vi "Build RT Data Cluster.vi"(0 "Device Reference in":T1 format="%.0x", 2 "RT Data in":T2={"Device ref"=0, "Scan Period (uSec)"=10000, "Device Channels"={"Status"={"BD Refs"=[], "Length"=0, "FIFO Index"=0, "Data"=[]}, "Command"={"BD Refs"=[], "Data"=[], "Length"=0, "FIFO Index"=0}}, "Local Chassis"=[], "EtherCAT Masters"=[], "Async"={"Status"=refnum, "Command"=refnum, "Input FIFO"=refnum, "Input FIFO buffer"=[], "Output FIFO"=refnum, "Output FIFO buffer"=[], "Async VI Ref"=refnum}, "ECAT Reconfig"={"Reconfig Module Found"=FALSE, "VI Ref"=refnum, "Status"=refnum}, "Device Error"={"status"=FALSE, "code"=0, "source"=""}, "DeviceName"="", "PCLSync?"=FALSE} {"Device Channels"."Status"."BD Refs"."Data Reference" format="%.0x"; "Device Channels"."Command"."BD Refs"."Data Reference" format="%.0x"; "Local Chassis"."FPGA"."VS ref" format="%.0x"; "Local Chassis"."RSI Modules"."VS ref" format="%.0x"; "Local Chassis"."VS ref" format="%.0x"; "Device ref" format="%.0x"; "EtherCAT Masters"."REM IO ECAT Slaves"."VS ref" format="%.0x"; "EtherCAT Masters"."Generic EtherCAT Slaves"."VS ref" format="%.0x"; "EtherCAT Masters"."VS ref" format="%.0x"; "EtherCAT Masters"."EtherCAT Slaves"."FPGA"."VS ref" format="%.0x"; "EtherCAT Masters"."EtherCAT Slaves"."RSI Modules"."VS ref" format="%.0x"; "EtherCAT Masters"."EtherCAT Slaves"."VS ref" format="%.0x"}, 3 "error in":errorcluster) -> (7 "RT Data out":T2={"Device ref"=0, "Scan Period (uSec)"=10000, "Device Channels"={"Status"={"BD Refs"=[], "Length"=0, "FIFO Index"=0, "Data"=[]}, "Command"={"BD Refs"=[], "Data"=[], "Length"=0, "FIFO Index"=0}}, "Local Chassis"=[], "EtherCAT Masters"=[], "Async"={"Status"=refnum, "Command"=refnum, "Input FIFO"=refnum, "Input FIFO buffer"=[], "Output FIFO"=refnum, "Output FIFO buffer"=[], "Async VI Ref"=refnum}, "ECAT Reconfig"={"Reconfig Module Found"=FALSE, "VI Ref"=refnum, "Status"=refnum}, "Device Error"={"status"=FALSE, "code"=0, "source"=""}, "DeviceName"="", "PCLSync?"=FALSE} {"Device Channels"."Status"."BD Refs"."Data Reference" format="%.0x"; "Device Channels"."Command"."BD Refs"."Data Reference" format="%.0x"; "Local Chassis"."FPGA"."VS ref" format="%.0x"; "Local Chassis"."RSI Modules"."VS ref" format="%.0x"; "Local Chassis"."VS ref" format="%.0x"; "Device ref" format="%.0x"; "EtherCAT Masters"."REM IO ECAT Slaves"."VS ref" format="%.0x"; "EtherCAT Masters"."Generic EtherCAT Slaves"."VS ref" format="%.0x"; "EtherCAT Masters"."VS ref" format="%.0x"; "EtherCAT Masters"."EtherCAT Slaves"."FPGA"."VS ref" format="%.0x"; "EtherCAT Masters"."EtherCAT Slaves"."RSI Modules"."VS ref" format="%.0x"; "EtherCAT Masters"."EtherCAT Slaves"."VS ref" format="%.0x"})   [LabVIEW 2020, in "SEECD Engine.lvlib"]
uses:
  SEECD Engine.lvlib
  Type Defs/RT Data.ctl
  <vilib>/NI VeriStand/Custom Device API/Custom Device Item Ref.ctl
  Type Defs/Device Channels.ctl
  Type Defs/Output Data.ctl
  <vilib>/NI VeriStand/Custom Device API/Block Data Reference.ctl
  <vilib>/NI VeriStand/Custom Device API/Data Reference.ctl
  Type Defs/Input Data.ctl
  Type Defs/Local Chassis Data.ctl
  Type Defs/RSI Module Data.ctl
  Type Defs/Open Module IOVs.ctl
  Includes/Modules.lvlibp/RSI Module/RSI Module.lvclass
  Includes/Modules.lvlibp/RSI Module/Module Models.ctl
  Includes/Modules.lvlibp/RSI Module/Channel Type.ctl
  Type Defs/Module Config Data.ctl
  Type Defs/Mixed IO.ctl
  Type Defs/FPGA Data.ctl
  Type Defs/UDV Data.ctl
  Shared/Type Defs/UDV Data Type.ctl
  Shared/Type Defs/FXP Config.ctl
  Type Defs/Mod Size Indexes.ctl
  Type Defs/EtherCAT Master Data.ctl
  Type Defs/EtherCAT Slave Data.ctl
  Type Defs/Generic ECAT Slave RT-Data-Array.ctl
  Type Defs/Generic ECAT Slave Data Cluster.ctl
  Type Defs/Generic ECAT Slave IOV Cluster.ctl
  Type Defs/REM IO ECAT Slave RT-Data-Array.ctl
  Type Defs/REM IO ECAT Slave Data Cluster.ctl
  Type Defs/REM IO ECAT Slave IOV Cluster.ctl
  Type Defs/Async Data.ctl
  Type Defs/Async Status.ctl
  Type Defs/Async State.ctl
  Type Defs/Async Command.ctl
  Type Defs/ECAT Reconfig Data.ctl
  Type Defs/ECAT Reconfig Status.ctl
  Type Defs/ECAT Reconfig State.ctl
  Type Defs/Data Ref FGV Command.ctl
  <vilib>/NIScanEngine/ConfigurableFaults/Fault Desc Control.ctl
  Shared/Globals/Property Strings.vi
  Shared/Globals/RT Globals.vi
  Shared/Globals/String Constants.vi
  <vilib>/NI VeriStand/Custom Device API/Get Item Property (U16).vi
  <vilib>/NI VeriStand/Custom Device API/Get Item Property (U32).vi
  <vilib>/NI VeriStand/Custom Device API/Custom Device API.lvlib
  Shared/SEECD Shared.lvlib
  <vilib>/NI VeriStand/Custom Device Tools/Custom Device Utility Library/Custom Device Utility Library.lvlib
  <vilib>/NIScanEngine/ConfigurableFaults/Config Faults.lvlib
  <vilib>/NI VeriStand/Custom Device API/Get Item Property (Boolean).vi
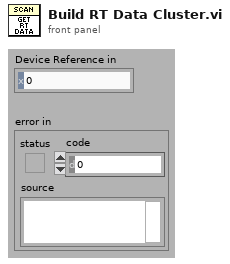
[diagram p1: front panel]
types:
  T1 = typedef "Custom Device API.lvlib/Custom Device Item Ref.ctl" = u64
  T2 = typedef "SEECD Engine.lvlib/RT Data.ctl" = cluster{"Device ref":T1, "Scan Period (uSec)":u32, "Device Channels":T3, "Local Chassis":T8[], "EtherCAT Masters":T20[], "Async":T28, "ECAT Reconfig":T29, "Device Error":errorcluster, "DeviceName":string, "PCLSync?":bool}
  T3 = typedef "SEECD Engine.lvlib/Device Channels.ctl" = cluster{"Status":T4, "Command":T7}
  T4 = typedef "SEECD Engine.lvlib/Output Data.ctl" = cluster{"BD Refs":T5[], "Length":i32, "FIFO Index":i32, "Data":dbl[]}
  T5 = typedef "Custom Device API.lvlib/Block Data Reference.ctl" = cluster{"Data Reference":T6, "Offset":u64, "Length":u64}
  T6 = typedef "Custom Device API.lvlib/Data Reference.ctl" = i32
  T7 = typedef "SEECD Engine.lvlib/Input Data.ctl" = cluster{"BD Refs":T5[], "Data":dbl[], "Length":i32, "FIFO Index":i32}
  T8 = typedef "SEECD Engine.lvlib/Local Chassis Data.ctl" = cluster{"VS ref":T1, "RSI Modules":T9[], "FPGA":T15[], "Input Mod Size Idxs":T19, "Output Modules":i32[], "MixedIO Mod Size Idxs":T19}
  T9 = typedef "SEECD Engine.lvlib/RSI Module Data.ctl" = cluster{"VS ref":T1, "IOV ref":refnum<k21>, "Open Mod refs":T10, "Module DVR":refnum<data-value>, "Slot":u32, "Model":T11, "Channel Type":T12, "EtherCAT?":bool, "CDInput Data":T7, "CDOutput Data":T4, "Module Config Data":T13, "Mixed IO":T14}
  T10 = typedef "SEECD Engine.lvlib/Open Module IOVs.ctl" = cluster{"Analog Read":refnum<k21>, "Digital Read":refnum<k21>, "Analog Write":refnum<k21>, "Digital Write":refnum<k21>}
  T11 = typedef "Modules.lvlibp/RSI Module.lvclass/Module Models.ctl" = enum16{"Empty", "NI 9201", "NI 9203", "NI 9205", "NI 9206", "NI 9207", "NI 9208", "NI 9209", "NI 9210", "NI 9211", "NI 9212", "NI 9213", "NI 9214", "NI 9215", "NI 9216", "NI 9217", "NI 9219", "NI 9220", "NI 9221", "NI 9222", "NI 9223", "NI 9224", "NI 9225", "NI 9226", "NI 9227", "NI 9228", "NI 9229", "NI 9233", "NI 9234", "NI 9235", "NI 9236", "NI 9237", "NI 9239", "NI 9242", "NI 9244", "NI 9253", "NI 9263", "NI 9264", "NI 9265", "NI 9266", "NI 9269", "NI 9344", "NI 9350", "NI 9375", "NI 9401", "NI 9402", "NI 9403", "NI 9411", "NI 9421", "NI 9422", "NI 9423", "NI 9425", "NI 9426", "NI 9435", "NI 9436", "NI 9437", "NI 9472", "NI 9474", "NI 9475", "NI 9476", "NI 9477", "NI 9478", "NI 9481", "NI 9482", "NI 9485"}
  T12 = typedef "Modules.lvlibp/RSI Module.lvclass/Channel Type.ctl" = enum16{"Analog", "Digital"}
  T13 = typedef "SEECD Engine.lvlib/Module Config Data.ctl" = cluster{"Configurable?":bool, "Config Block Data Refs":T5[], "Config Data DVR":refnum<data-value>, "Previous Values":dbl[], "Local Reconfig VI Ref":refnum<vi>}
  T14 = typedef "SEECD Engine.lvlib/Mixed IO.ctl" = cluster{"Input Channel Indices":i32[], "Input Buffer":dbl[]}
  T15 = typedef "SEECD Engine.lvlib/FPGA Data.ctl" = cluster{"VS ref":T1, "IOV ref":refnum<k21>, "FPGA Target":enum16{"Local", "EtherCAT"}, "Product Code":u32, "Bitfile Signature":string, "Bitfile Path (RT)":path, "FPGA Session":u32, "Input Data":T7, "Output Data":T4, "UDVs":cluster{"From FPGA":T16[], "To FPGA":T16[]}}
  T16 = typedef "SEECD Engine.lvlib/UDV Data.ctl" = cluster{"VS ref":T1, "IOV Ref":refnum<k21>, "Name":string, "UDV Data Type":T17, "Supported Type?":bool, "FXP Config":T18, "FXP VI Ref":refnum<vi>}
  T17 = typedef "SEECD Shared.lvlib/UDV Data Type.ctl" = enum16{"Boolean", "Fixed Point", "Int8", "Int16", "Int32", "Int64", "U32 Bit Field", "UInt8", "UInt16", "UInt32", "UInt64", "Other", "DBL", "SGL"}
  T18 = typedef "SEECD Shared.lvlib/FXP Config.ctl" = cluster{"signed":bool, "size":u32, "integersize":i32}
  T19 = typedef "SEECD Engine.lvlib/Mod Size Indexes.ctl" = cluster{"4":i32[], "8":i32[], "16":i32[], "32":i32[], "other":i32[]}
  T20 = typedef "SEECD Engine.lvlib/EtherCAT Master Data.ctl" = cluster{"VS ref":T1, "IOV ref":refnum<k21>, "Master ID":u32, "Cyclic Data Bandwidth":u32, "EtherCAT Slaves":T21[], "Generic EtherCAT Slaves":T22, "REM IO ECAT Slaves":T25}
  T21 = typedef "SEECD Engine.lvlib/EtherCAT Slave Data.ctl" = cluster{"VS ref":T1, "IOV ref":refnum<k21>, "Position Address":u16, "RSI Modules":T9[], "FPGA":T15[], "Input Mod Size Idxs":T19, "Output Modules":i32[], "MixedIO Mod Size Idxs":T19}
  T22 = typedef "SEECD Engine.lvlib/Generic ECAT Slave RT-Data-Array.ctl" = T23[]
  T23 = typedef "SEECD Engine.lvlib/Generic ECAT Slave Data Cluster.ctl" = cluster{"VS ref":T1, "IOV ref":refnum<k21>, "Position Address":u16, "I/O Imput Vars ":T24[], "I/O Output Vars":T24[], "I/O Input Data":T7, "I/O Output Data":T4, "Distributed Clock":bool}
  T24 = typedef "SEECD Engine.lvlib/Generic ECAT Slave IOV Cluster.ctl" = cluster{"VS ref":T1, "IOV Ref":refnum<k21>, "Name":string, "UDV Data Type":T17}
  T25 = typedef "SEECD Engine.lvlib/REM IO ECAT Slave RT-Data-Array.ctl" = T26[]
  T26 = typedef "SEECD Engine.lvlib/REM IO ECAT Slave Data Cluster.ctl" = cluster{"VS ref":T1, "IOV ref":refnum<k21>, "Position Address":u16, "I/O Imput Vars ":T27[], "I/O Output Vars":T27[], "I/O Input Data":T7, "I/O Output Data":T4}
  T27 = typedef "SEECD Engine.lvlib/REM IO ECAT Slave IOV Cluster.ctl" = cluster{"VS ref":T1, "IOV Ref":refnum<k21>, "Name":string, "UDV Data Type":T17, "Scaling Factor":dbl}
  T28 = typedef "SEECD Engine.lvlib/Async Data.ctl" = cluster{"Status":refnum<queue>, "Command":refnum<queue>, "Input FIFO":refnum<k33>, "Input FIFO buffer":dbl[], "Output FIFO":refnum<k33>, "Output FIFO buffer":dbl[], "Async VI Ref":refnum<vi>}
  T29 = typedef "SEECD Engine.lvlib/ECAT Reconfig Data.ctl" = cluster{"Reconfig Module Found":bool, "VI Ref":refnum<vi>, "Status":refnum<queue>}
  T30 = typedef "Config Faults.lvlib/Fault Desc Control.ctl" = cluster{"code":i32, "level or level before threshold":i32, "occurrence threshold":u32, "time window in seconds":u32, "level after threshold":i32}
  T31 = typedef "SEECD Engine.lvlib/Data Ref FGV Command.ctl" = enum16{"Intialize", "Get", "Update"}
  T32 = typedef "Fault.ctl" = cluster{"code":i32, "level":i32, "first reported time":timestamp, "number reported":u32}
  T33 = typedef "Custom Device API.lvlib/Custom Device Channel.ctl" = cluster{"Type":T34, "Units":string, "Default Value":dbl, "Faultable":bool, "Scalable":bool}
  T34 = typedef "Custom Device API.lvlib/Custom Device Channel Type.ctl" = enum16{"Input", "Output"}
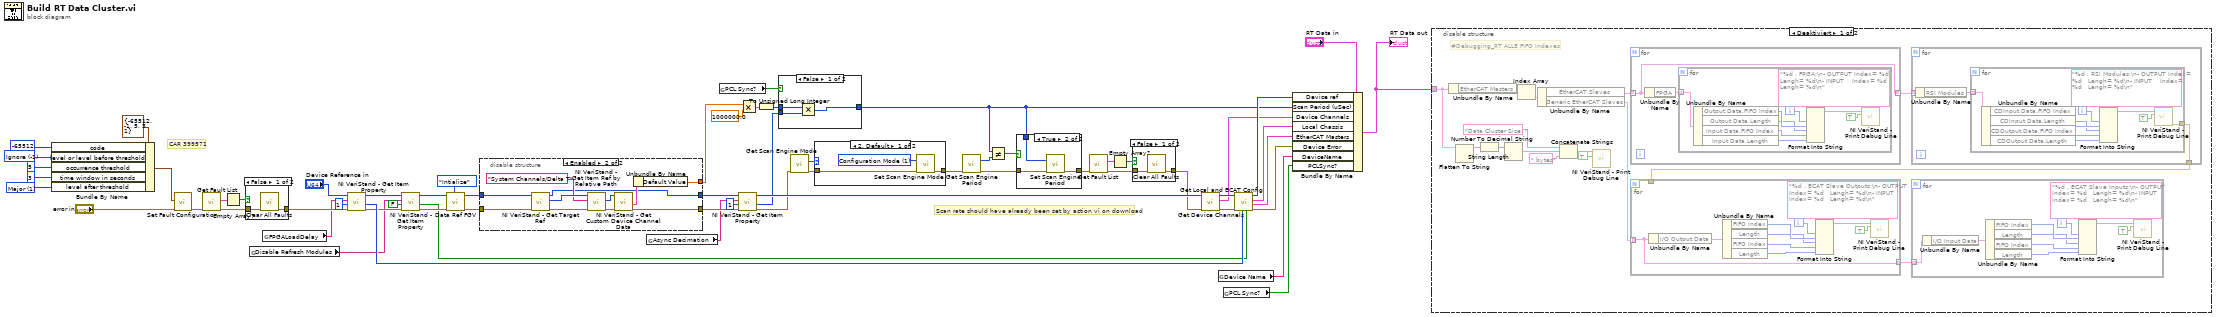
[diagram p0: block diagram]
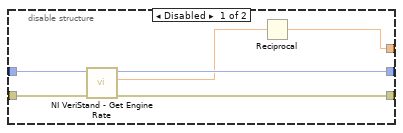
[diagram p7: hidden frame]
diagram:
  w19 = -1 items=["Ignore"=-1, "Minor"=0, "Major"=1] ("level or level before threshold")
  w22 = 1 items=["Ignore"=-1, "Minor"=0, "Major"=1] ("level after threshold")
  # "CAR 399571"
  # "Scan rate should have already been set by action vi on download"
  n1 = Bundle By Name(cluster=T30 {"code"=-65512, "level or level before threshold"=-1, "occurrence threshold"=5, "time window in seconds"=3, "level after threshold"=1} ("fault configuration"), "code"=-65512, "level or level before threshold"=w19, "occurrence threshold"=u32 5, "time window in seconds"=u32 3, "level after threshold"=w22) -> (w23:T30)
  n2 = call <vilib>:"Set Fault Configuration.vi"("error in (no error)"="error in", "fault configuration"=w23) -> ("error out"=w17:errorcluster)  [unwired: 7 in]
  n3 = call <vilib>:"Get Fault List.vi"("error in (no error)"=w17) -> ("error out"=w28:errorcluster, "fault list"=w26:T32[])  [unwired: 9 in]
  n4 = Empty Array?(array=w26) -> (empty?=w27:bool)
  n5 = case shown="False" w27 {
    tunnel: w28 -> [w64 w65]
    tunnel: [w63 w65] -> w25
    frame False {
      n6 = call <vilib>:"Clear All Faults.vi"("error in (no error)"=w64) -> ("error out"=w63:errorcluster)  [unwired: 10 in]
    }
    frame True {
    }
  }
  n7 = global read "Property Strings.vi" "Disable Refresh Modules"() -> (w3:string)
  n8 = global read "Property Strings.vi" "FPGALoadDelay"() -> (w12:string)
  n9 = call-poly <vilib>:"NI VeriStand - Get Item Property.vi"("error in (no error)"=w25, "Default Value"=u16 1, "Property Name"=w12, "Item Ref in"="Device Reference in") -> ("error out"=w7:errorcluster, "Value"=w9:u16, "Item Ref out"=w5:T1)  [unwired: 4 in, 1 out]
  n10 = call-poly <vilib>:"NI VeriStand - Get Item Property.vi"("error in (no error)"=w7, "Default Value"=FALSE, "Property Name"=w3, "Item Ref in"=w5) -> ("error out"=w6:errorcluster, "Value"=w1:bool, "Item Ref out"=w4:T1)  [unwired: 4 in, 1 out]
  n11 = call "Data Ref FGV.vi"("Command"=Data_Ref_FGV_Command."Intialize", "error in (no error)"=w6, "Device Ref in"=w4) -> ("error out"=w62:errorcluster, "Device Ref out"=w61:T1)  [unwired: 5 in, 2 out]
  n12 = disable-structure shown="Enabled" {
    disable-tunnel: [w66 w73] -> w56
    disable-tunnel: [w71 w72] -> w50
    disable-tunnel: [w70 w74] -> w51
    disable-tunnel: w62 -> [w69 w81]
    disable-tunnel: w61 -> [w68 w82]
    frame Disabled {
      n13 = call <vilib>:"NI VeriStand - Get Engine Rate.vi"("error in (no error)"=w69, "Item Ref in"=w68) -> ("error out"=w71:errorcluster, "Rate (Hz)"=w67:dbl, "Item Ref out"=w70:T1)  [unwired: 7 in]
      n14 = Reciprocal(x=w67) -> (1/x=w66:dbl)
    }
    frame Enabled {
      n15 = call <vilib>:"NI VeriStand - Get Target Ref.vi"("error in"=w81, "Item Ref in"=w82) -> ("error out"=w79:errorcluster, "Target Ref"=w80:T1, "Item Ref out"=w74:T1)  [unwired: 6 in, 1 out]
      n16 = call <vilib>:"NI VeriStand - Get Item Ref by Relative Path.vi"("error in"=w79, "Relative Item Path"="System Channels/Delta T", "Section Ref in"=w80) -> ("error out"=w76:errorcluster, "Item Ref"=w77:T1)  [unwired: 5 in, 2 out]
      n17 = call <vilib>:"NI VeriStand - Get Custom Device Channel Data.vi"("error in (no error)"=w76, "Channel Ref in"=w77) -> ("error out"=w72:errorcluster, "Channel"=w75:T33)  [unwired: 4 in, 4 out]
      n18 = Unbundle By Name(w75) -> ("Default Value"=w73:dbl)
    }
  }
  n19 = global read "Property Strings.vi" "Async Decimation"() -> (w48:string)
  n20 = global read "RT Globals.vi" "PCL Sync?"() -> (w45:bool)
  n21 = call-poly <vilib>:"NI VeriStand - Get Item Property.vi"("error in (no error)"=w50, "Default Value"=u32 1, "Property Name"=w48, "Item Ref in"=w51) -> ("error out"=w36:errorcluster, "Value"=w46:u32, "Item Ref out"=w49:T1)  [unwired: 4 in, 1 out]
  n22 = Multiply(x=w56, y=1000000.0) -> (x*y=w30:dbl)
  n23 = To Unsigned Long Integer(number=w30) -> (unsigned 32bit integer=w29:u32)
  n24 = case shown="False" w45 {
    tunnel: w29 -> [w85 w86]
    tunnel: w46 -> [w84 _]
    tunnel: [w83 w86] -> w31
    frame False {
      n25 = Multiply(x=w85, y=w84) -> (x*y=w83:u32)
    }
    frame True {
    }
  }
  n26 = call <vilib>:"Get Scan Engine Mode.vi"("error in (no error)"=w36) -> ("error out"=w38:errorcluster, "mode"=w37:i32)  [unwired: 9 in]
  n27 = case shown="2, Default" w37 {
    tunnel: w38 -> [w88 w90]
    tunnel: [w87 w90] -> w35
    frame 2, Default {
      w89 = 1 items=["Configuration Mode"=1, "Active Mode"=2] ("mode (Active Mode)")
      n28 = call <vilib>:"Set Scan Engine Mode.vi"("mode (Active Mode)"=w89, "error in (no error)"=w88) -> ("error out"=w87:errorcluster)  [unwired: 13 in]
    }
    frame 1 {
    }
  }
  n29 = call <vilib>:"Get Scan Engine Period.vi"("error in (no error)"=w35) -> ("scan period (uSec)"=w34:u32, "error out"=w32:errorcluster)  [unwired: 13 in]
  n30 = Not Equal?(x=w31, y=w34) -> (x != y?=w33:bool)
  n31 = case shown="True" w33 {
    tunnel: [w91 w94] -> w40
    tunnel: w32 -> [w91 w93]
    tunnel: w31 -> [_ w92]
    frame False {
    }
    frame True {
      n32 = call <vilib>:"Set Scan Engine Period.vi"("scan period (uSec)"=w92, "error in (no error)"=w93) -> ("error out"=w94:errorcluster)  [unwired: 13 in]
    }
  }
  n33 = call <vilib>:"Get Fault List.vi"("error in (no error)"=w40) -> ("error out"=w43:errorcluster, "fault list"=w41:T32[])  [unwired: 9 in]
  n34 = Empty Array?(array=w41) -> (empty?=w42:bool)
  n35 = case shown="False" w42 {
    tunnel: w43 -> [w96 w97]
    tunnel: [w95 w97] -> w39
    frame False {
      n36 = call <vilib>:"Clear All Faults.vi"("error in (no error)"=w96) -> ("error out"=w95:errorcluster)  [unwired: 10 in]
    }
    frame True {
    }
  }
  n37 = call "Get Device Channels.vi"("error in"=w39, "Device Reference in"=w49) -> ("error out"=w54:errorcluster, "Device Channels"=w52:T3, "Device Reference out"=w53:T1)  [unwired: 7 in]
  n38 = global read "String Constants.vi" "Device Name"() -> (w15:string)
  n39 = global read "RT Globals.vi" "PCL Sync?"() -> (w14:bool)
  n40 = call "Get Local and ECAT Config.vi"("Disable Refresh Modules"=w1, "fpga wait (s)"=w9, "error in (no error)"=w54, "Device Reference in"=w53) -> ("error out"=w10:errorcluster, "ECAT Masters"=w44:T20[], "Local Chassis"=w60:T8[], "Device Reference out"=w58:T1)  [unwired: 4 in]
  n41 = Bundle By Name(cluster="RT Data in", "Device ref"=w58, "Scan Period (uSec)"=w31, "Device Channels"=w52, "Local Chassis"=w60, "EtherCAT Masters"=w44, "Device Error"=w10, "DeviceName"=w15, "PCLSync?"=w14) -> (w8:T2)
  "RT Data out" <- w8
  n42 = disable-structure shown="Deaktiviert" {
    disable-tunnel: w8 -> [w100 _]
    frame Disabled {
      # "#Debugging_RT ALLE FIFO Indexes"
      n43 = Unbundle By Name(w100) -> ("EtherCAT Masters"=w112:T20[])
      n44 = Flatten To String(anything=w100) -> (data string=w105:string)  [unwired: 3 in, 2 out]
      n45 = String Length(string=w105) -> (length=w103:i32)
      n46 = Number To Decimal String(number=w103) -> (decimal integer string=w102:string)  [unwired: 1 in]
      n47 = Index Array(array=w112) -> (element=w111:T20)  [unwired: 1 in]
      n48 = Unbundle By Name(w111) -> ("EtherCAT Slaves"=w110:T21[], "Generic EtherCAT Slaves"=w108:T22)
      n49 = Concatenate Strings("Data Cluster Size: " ("string"), w102, " bytes" ("string")) -> (w99:string)
      n50 = call <vilib>:"NI VeriStand - Print Debug Line.vi"("Add to log file? (F)"=TRUE, "Message"=w99) -> ()  [unwired: 9 in, 1 out]
      n51 = for {
        tunnel: w110 -> [w146] mode=indexing
        tunnel: [w146] -> w109 mode=indexing
        n52 = Unbundle By Name(w146) -> ("FPGA"=w147:T15[])
        n53 = for {
          tunnel: w147 -> [w156] mode=indexing
          i -> [w152]
          n54 = Unbundle By Name(w156) -> ("Output Data.FIFO Index"=w151:i32, "Output Data.Length"=w150:i32, "Input Data.FIFO Index"=w149:i32, "Input Data.Length"=w148:i32)
          n55 = Format Into String(format string="%d . FPGA:\n- OUTPUT Index= %d   Lengh= %d\n- INPUT    Index= %d   Lengh= %d\n", w152, w151, w150, w149, w148) -> (resulting string=w155:string)  [unwired: 2 in, 1 out]
          n56 = call <vilib>:"NI VeriStand - Print Debug Line.vi"("Add to log file? (F)"=TRUE, "Message"=w155) -> ()  [unwired: 9 in, 1 out]
        }
      }
      n57 = for {
        tunnel: w109 -> [w134] mode=indexing
        tunnel: [w133] -> w106
        n58 = Unbundle By Name(w134) -> ("RSI Modules"=w135:T9[])
        n59 = for {
          tunnel: w135 -> [w145] mode=indexing
          tunnel: [w137] -> w133
          i -> [w142]
          n60 = Unbundle By Name(w145) -> ("CDInput Data.FIFO Index"=w141:i32, "CDInput Data.Length"=w140:i32, "CDOutput Data.FIFO Index"=w139:i32, "CDOutput Data.Length"=w138:i32)
          n61 = Format Into String(format string="%d . RSI Modules:\n- OUTPUT Index= %d   Lengh= %d\n- INPUT    Index= %d   Lengh= %d\n", w142, w141, w140, w139, w138) -> (resulting string=w144:string)  [unwired: 2 in, 1 out]
          n62 = call <vilib>:"NI VeriStand - Print Debug Line.vi"("Add to log file? (F)"=TRUE, "Message"=w144) -> ("error out"=w137:errorcluster)  [unwired: 9 in]
        }
      }
      n63 = for {
        tunnel: w108 -> [w124] mode=indexing
        tunnel: [w124] -> w107 mode=indexing
        tunnel: w106 -> [_]
        i -> [w130]
        n64 = Unbundle By Name(w124) -> ("I/O Output Data"=w125:T4)
        n65 = Unbundle By Name(w125) -> ("FIFO Index"=w129:i32, "Length"=w128:i32, "FIFO Index"=w127:i32, "Length"=w126:i32)
        n66 = Format Into String(format string="%d . ECAT Slave Outputs:\n- OUTPUT Index= %d   Lengh= %d\n- INPUT    Index= %d   Lengh= %d\n", w130, w129, w128, w127, w126) -> (resulting string=w132:string)  [unwired: 2 in, 1 out]
        n67 = call <vilib>:"NI VeriStand - Print Debug Line.vi"("Add to log file? (F)"=TRUE, "Message"=w132) -> ()  [unwired: 9 in, 1 out]
      }
      n68 = for {
        tunnel: w107 -> [w114] mode=indexing
        i -> [w120]
        n69 = Unbundle By Name(w114) -> ("I/O Input Data"=w115:T7)
        n70 = Unbundle By Name(w115) -> ("FIFO Index"=w119:i32, "Length"=w118:i32, "FIFO Index"=w117:i32, "Length"=w116:i32)
        n71 = Format Into String(format string="%d . ECAT Slave Inputs:\n- OUTPUT Index= %d   Lengh= %d\n- INPUT    Index= %d   Lengh= %d\n", w120, w119, w118, w117, w116) -> (resulting string=w122:string)  [unwired: 2 in, 1 out]
        n72 = call <vilib>:"NI VeriStand - Print Debug Line.vi"("Add to log file? (F)"=TRUE, "Message"=w122) -> ()  [unwired: 9 in, 1 out]
      }
    }
    frame Enabled {
    }
  }
